vi "Make Log Directory.vi"(8 "error in (no error)":errorcluster, 11 "File Handler in":refnum<class "File Handler.lvclass">) -> (0 "error out":errorcluster, 3 "dup File Handler":refnum<class "File Handler.lvclass">)   [LabVIEW 2018, in "GLog.lvlib" / "File Handler.lvclass"]
uses:
  File Handler.lvclass
  File Handler.lvclass/File Handler.ctl
panel:
  # "Connector Pane"
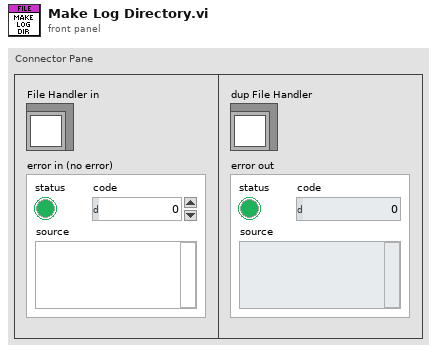
[diagram p1: front panel]
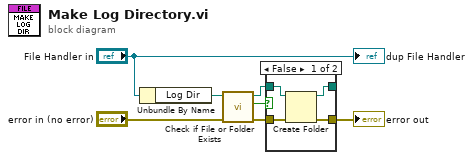
[diagram p0: block diagram]
diagram:
  n1 = Unbundle By Name("File Handler in") -> ("Log Dir"=w1:path)
  n2 = call <vilib>:"Check if File or Folder Exists.vi"("error in (no error)"="error in (no error)", "path"=w1) -> ("error out"=w3:errorcluster, "file or folder exists?"=w4:bool, "dup path"=w5:path)  [unwired: 7 in]
  n3 = case shown="False" w4 {
    tunnel: [w9 w13] -> w2
    tunnel: w3 -> [w11 w13]
    tunnel: w5 -> [w10 w12]
    tunnel: [w8 w12] -> _
    frame False {
      n4 = Create Folder(path (use dialog)=w10, error in=w11) -> (created path=w8:path, error out=w9:errorcluster)  [unwired: 1 in, 1 out]
    }
    frame True {
    }
  }
  "error out" <- w2
  "dup File Handler" <- "File Handler in"
